vi "UpdateDependency.vi"(8 "error in (no error)":errorcluster, 10 "Dependency":variant, 11 "Provider in":refnum<class "Provider.lvclass">) -> (0 "error out":errorcluster, 3 "Provider out":refnum<class "Provider.lvclass">)   [LabVIEW 2024, in "Provider.lvclass"]
uses:
  Provider.lvclass
  Provider.lvclass/Provider.ctl
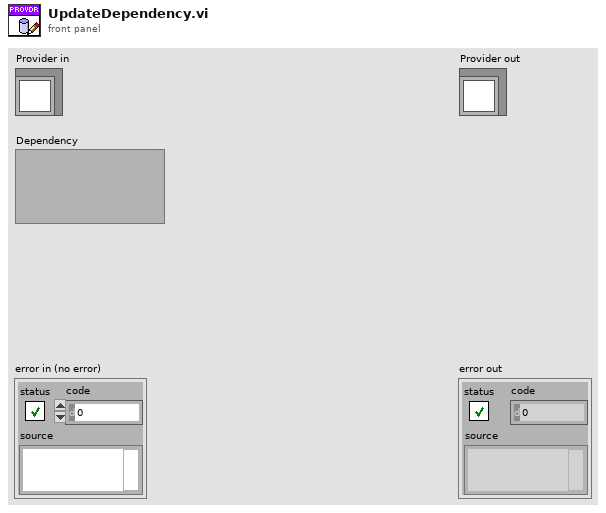
[diagram p1: front panel]
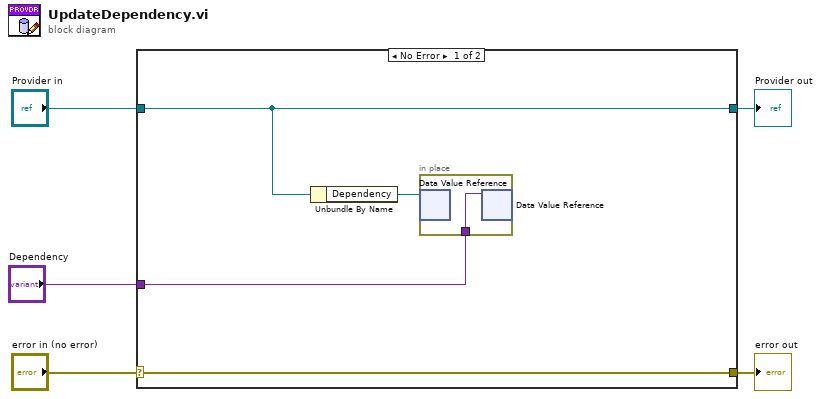
[diagram p0: block diagram]
diagram:
  n1 = case shown="No Error" "error in (no error)" {
    selector: "error in (no error)" -> [w9 w12]
    tunnel: [w9 w12] -> w4
    tunnel: [w8 w11] -> w2
    tunnel: "Provider in" -> [w8 w11]
    tunnel: "Dependency" -> [w6 _]
    frame No Error {
      n2 = Unbundle By Name(w8) -> ("Dependency"=w7:refnum<data-value>)
      n3 = in-place {
        in-place-border: w6 -> [w10]
        n4 = in-place-dvr #1(w7) -> ()  [unwired: 2 out]
        n5 = in-place-dvr #1(w10) -> ()  [unwired: 2 out]
      }
    }
    frame Error {
    }
  }
  "error out" <- w4
  "Provider out" <- w2
